vi "Legacy Cancellations.vi"(8 "error in":errorcluster, 9 "started id":string, 10 "add?":bool, 11 "request id":string) -> (0 "error out":errorcluster, 3 "recorded?":bool)   [LabVIEW 2020, in "MCP Server.lvlib"]
doc: "Functional global that remembers the request ids named by legacy notifications/cancelled messages (MCP 2025-06-18 and older: the client POSTs {\"method\":\"notifications/cancelled\",\"params\":{\"requestId\":..}}), at most 16 of them. Prepare Request Dispatch.vi records them before Handle MCP Request.vi runs; Report Progress.vi and Cancel Requested.vi ask whether the id of the running request is among them.\n\nstarted id: Prepare Request Dispatch.vi passes the id of every request it dispatches. That id is forgotten first, so a cancellation that arrived too late (after its request had finished) never cancels a later request that reuses the id.\nadd? TRUE then records request id. recorded? is TRUE when request id is among the remembered ids. Ids are compared as JSON text (5 and \"5\" are different ids, as in JSON-RPC). An empty id or null is never recorded."
uses:
  MCP Server.lvlib
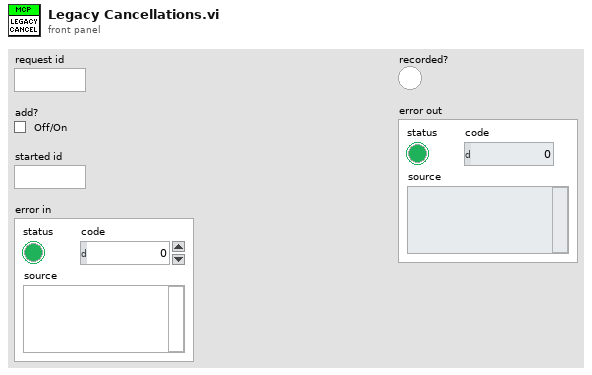
[diagram p1: front panel]
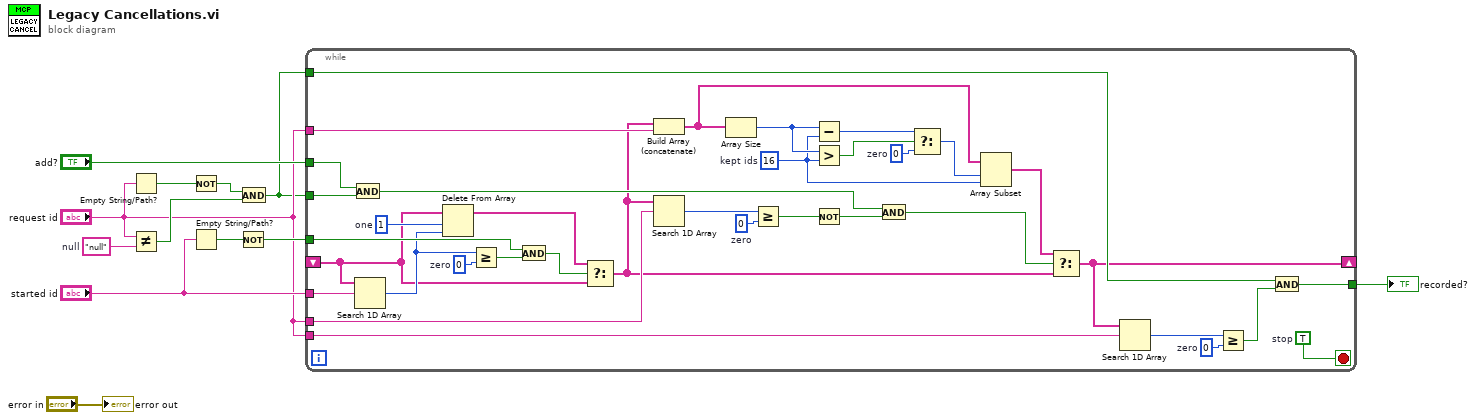
[diagram p0: block diagram]
diagram:
  w11 = "null"  # null
  n1 = Empty String/Path?(string/path="request id") -> (empty?=w12:bool)
  n2 = Not Equal?(x="request id", y=w11) -> (x != y?=w9:bool)
  n3 = Not(x=w12) -> (.not. x?=w10:bool)
  n4 = Empty String/Path?(string/path="started id") -> (empty?=w8:bool)
  n5 = Not(x=w8) -> (.not. x?=w6:bool)
  n6 = And(x=w10, y=w9) -> (x .and. y?=w3:bool)
  n7 = while {
    tunnel: "started id" -> [w48]
    tunnel: w6 -> [w46]
    tunnel: "request id" -> [w40]
    tunnel: "request id" -> [w37]
    tunnel: "add?" -> [w29]
    tunnel: w3 -> [w28]
    tunnel: "request id" -> [w21]
    tunnel: w3 -> [w18]
    shift-right: [w16] -> _
    shift-left: _ -> [w15]
    tunnel: [w13] -> w2
    stop <- w14 stop-if-true
    w14 = TRUE  # stop
    w19 = 0  # zero
    w33 = 0  # zero
    w30 = 16  # kept ids
    w38 = 0  # zero
    w44 = 1  # one
    w47 = 0  # zero
    n8 = And(x=w29, y=w28) -> (x .and. y?=w26:bool)
    n9 = Search 1D Array(1D array=w15, element=w48) -> (index of element=w43:i32)  [unwired: 1 in]
    n10 = Delete From Array(array=w15, length=w44, index=w43) -> (array with subset deleted=w42:string[])  [unwired: 1 out]
    n11 = Greater Or Equal?(x=w43, y=w47) -> (x >= y?=w45:bool)
    n12 = And(x=w46, y=w45) -> (x .and. y?=w41:bool)
    n13 = Select(t=w42, s=w41, f=w15) -> (s? t:f=w22:string[])
    n14 = Build Array (concatenate)(w22, w37) -> (w32:string[])
    n15 = Search 1D Array(1D array=w22, element=w40) -> (index of element=w39:i32)  [unwired: 1 in]
    n16 = Array Size(array=w32) -> (size(s)=w36:i32)
    n17 = Greater Or Equal?(x=w39, y=w38) -> (x >= y?=w27:bool)
    n18 = Subtract(x=w36, y=w30) -> (x-y=w35:i32)
    n19 = Greater?(x=w36, y=w30) -> (0:w34:bool)
    n20 = Not(x=w27) -> (.not. x?=w25:bool)
    n21 = And(x=w26, y=w25) -> (x .and. y?=w23:bool)
    n22 = Select(t=w35, s=w34, f=w33) -> (s? t:f=w31:i32)
    n23 = Array Subset(array=w32, index=w31, length=w30) -> (w24:string[])
    n24 = Select(t=w24, s=w23, f=w22) -> (s? t:f=w16:string[])
    n25 = Search 1D Array(1D array=w16, element=w21) -> (index of element=w20:i32)  [unwired: 1 in]
    n26 = Greater Or Equal?(x=w20, y=w19) -> (x >= y?=w17:bool)
    n27 = And(x=w18, y=w17) -> (x .and. y?=w13:bool)
  }
  "recorded?" <- w2
  "error out" <- "error in"
